vi "RemoteVI Complex Fixture Find Controls.vi"(0 "Panel":refnum<vi>, 5 "labels":string[](array[string]), 11 "error in":errorcluster) -> (4 "Controls":refnum<vi>[](array[refnum]), 15 "error out":errorcluster)   [LabVIEW 2020]
doc: "Helper of RemoteVI Complex Fixture.vi. Returns a reference to the control labelled each of labels, searched among all controls RemoteVI Complex Fixture All Controls.vi finds on Panel (every pane, tab pages, clusters), in the order of labels; Not a Refnum for a label no control carries. For registering the events of controls pasted in after generation. Errors of the property reads go to error out."
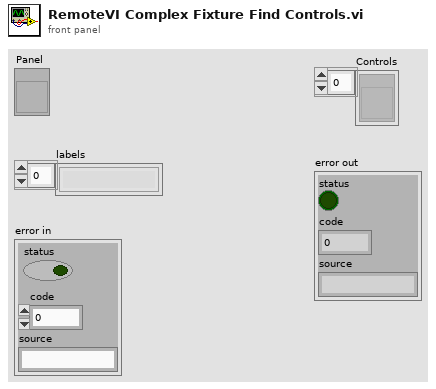
[diagram p1: front panel]
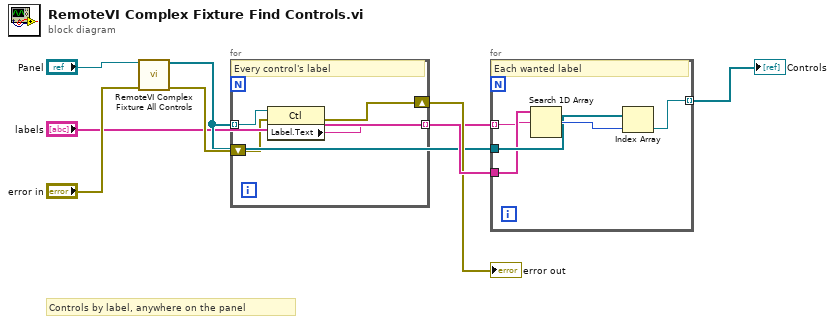
[diagram p0: block diagram]
diagram:
  # "Controls by label, anywhere on the panel"
  n1 = call "RemoteVI Complex Fixture All Controls.vi"("Panel"="Panel", "error in"="error in") -> ("Controls"=w4:refnum<vi>[], "error out"=w5:errorcluster)  [unwired: 12 in]
  n2 = for {
    tunnel: w4 -> [w9] mode=indexing
    shift-right: [w11] -> w6
    shift-left: w5 -> [w10]
    tunnel: [w12] -> w7 mode=indexing
    # "Every control's label"
    n3 = property class="Ctl"(reference=w9, error in=w10) -> (error out=w11:errorcluster, "Label.Text"=w12:string)  [unwired: 1 out]
  }
  "error out" <- w6
  n4 = for {
    tunnel: "labels" -> [w13] mode=indexing
    tunnel: w4 -> [w15]
    tunnel: w7 -> [w14]
    tunnel: [w17] -> w8 mode=indexing
    # "Each wanted label"
    n5 = Search 1D Array(1D array=w14, element=w13) -> (index of element=w16:i32)  [unwired: 1 in]
    n6 = Index Array(array=w15, index=w16) -> (element=w17:refnum<vi>)
  }
  "Controls" <- w8
